vi "SlewRateLimiter_Execute.vi"(6 "Enable":bool=TRUE, 8 "Time":dbl=-1.0 format="%33.4f", 9 "NegativeRate":dbl=1.0, 10 "PositiveRate":dbl, 11 "Input":dbl) -> (1 "Output":dbl, 3 "out SLEW_RATE_LIMITER":T1 {"NegativeRateLimit" format="%13.5p"; "PrevTime" format="%30.5p"; "PrevValue" format="%13.5p"; "PositiveRateLimit" format="%13.5p"})   [LabVIEW 2019, in "Trajectory_Library.lvlib"]
doc: "Convience, single call, LabVIEW function. Creates and calculates the slew rate limiter function to filter the input to limit its slew rate. The optional enable parameter bypasses the filter calculation when \"enabled\" is false. When enabled is \"false\" the input is passed directly to the output and the internal buffer is continually filled with the current input value.\n\n\nThis limits the rate of change of an input value. Useful for implementing voltage, setpoint, and/or output ramps. A slew-rate limit is most appropriate when the quantity being controlled is a velocity or a voltage; when controlling a position, consider using a postion control algoritmn or trapezoid profile instead.\n\nInputs:\n - input -- The input value whose slew rate is to be limited.\n - Positive Rate -- The new positive rate limit in units/second. This is expected to be >= 0.\n - Negative Rate -- The new negative rate limit in units/second. This is expected to be <= 0. Optional. If not wired or the value is > 0 then the Positive Rate * -1 is used.\n - enable -- Perform the rate limit calcuation when True. When False, output the input value unchanged. (Default=True)\n\nOutputs:\n - out Slew Rate Limiter -- The modified Slew Rate Limiter data cluster\n - output -- The filtered value, which will not change faster than the slew rate."
uses:
  Trajectory_Library.lvlib
  TypeDef/SLEW_RATE_LIMITER.ctl
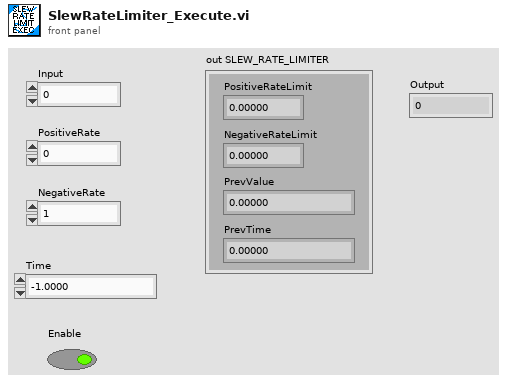
[diagram p1: front panel]
types:
  T1 = typedef "Trajectory_Library.lvlib/SLEW_RATE_LIMITER.ctl" = cluster{"PositiveRateLimit":dbl, "PrevValue":dbl, "PrevTime":dbl, "NegativeRateLimit":dbl}
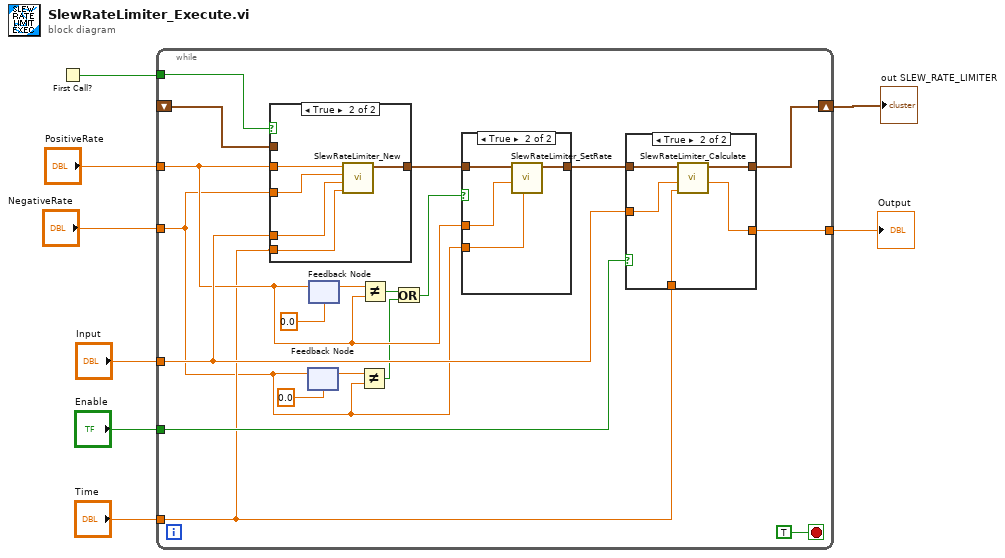
[diagram p0: block diagram]
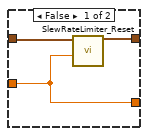
[diagram p3: hidden frame]
diagram:
  n1 = First Call?() -> (First Call?: T/F=w8:bool)
  n2 = while {
    tunnel: w8 -> [w27]
    tunnel: [w25] -> w6
    tunnel: "Enable" -> [w24]
    tunnel: "Input" -> [w23]
    tunnel: "PositiveRate" -> [w20]
    tunnel: "Time" -> [w17]
    shift-right: [w26] -> w7
    shift-left: _ -> [w15]
    tunnel: "NegativeRate" -> [w9]
    stop <- TRUE stop-if-true
    n3 = case shown="True" w27 {
      tunnel: [w41 w46] -> w22
      tunnel: w15 -> [w41 _]
      tunnel: w20 -> [_ w45]
      tunnel: w23 -> [_ w44]
      tunnel: w17 -> [_ w43]
      tunnel: w9 -> [_ w42]
      frame False {
      }
      frame True {
        n4 = call "SlewRateLimiter_New.vi"("Time"=w43, "InitialValue"=w44, "NegativeRateLimit"=w42, "PositiveRateLimit"=w45) -> ("out SLEW_RATE_LIMITER"=w46:T1)  [unwired: 7 in]
      }
    }
    n5 = feedback #1(0.0 ("Rate")) -> (w14:dbl)
    n6 = feedback-in #1(w9) -> ()
    n7 = feedback #2(0.0 ("Rate")) -> (w21:dbl)
    n8 = feedback-in #2(w20) -> ()
    n9 = Not Equal?(x=w14, y=w9) -> (x != y?=w10:bool)
    n10 = Not Equal?(x=w21, y=w20) -> (x != y?=w12:bool)
    n11 = Or(x=w12, y=w10) -> (x .or. y?=w11:bool)
    n12 = case shown="True" w11 {
      tunnel: w22 -> [w28 w31]
      tunnel: [w28 w32] -> w18
      tunnel: w20 -> [_ w30]
      tunnel: w9 -> [_ w29]
      frame False {
      }
      frame True {
        n13 = call "SlewRateLimiter_SetRate.vi"("NegativeRate"=w29, "PositiveRate"=w30, "in SLEW_RATE_LIMITER"=w31) -> ("out SLEW_RATE_LIMITER"=w32:T1)  [unwired: 8 in]
      }
    }
    n14 = case shown="True" w24 {
      tunnel: w18 -> [w35 w40]
      tunnel: [w33 w39] -> w26
      tunnel: [w34 w38] -> w25
      tunnel: w23 -> [w34 w37]
      tunnel: w17 -> [_ w36]
      frame False {
        n15 = call "SlewRateLimiter_Reset.vi"("ResetValue"=w34, "in SLEW_RATE_LIMITER"=w35) -> ("out SLEW_RATE_LIMITER"=w33:T1)  [unwired: 9 in]
      }
      frame True {
        n16 = call "SlewRateLimiter_Calculate.vi"("Time"=w36, "Input"=w37, "in SLEW_RATE_LIMITER"=w40) -> ("Output"=w38:dbl, "out SLEW_RATE_LIMITER"=w39:T1)  [unwired: 7 in]
      }
    }
  }
  "out SLEW_RATE_LIMITER" <- w7
  "Output" <- w6
